vi "Untitled 2.vi"() -> ()   [LabVIEW 2023]
panel:
  out "error in (no error) 2":errorcluster
  in  "error in (no error)":errorcluster
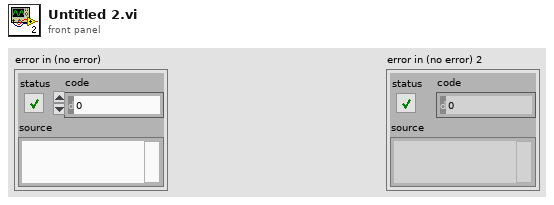
[diagram p1: front panel]
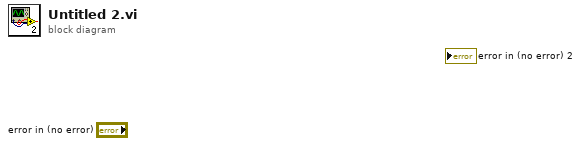
[diagram p0: block diagram]
diagram:
